vi "Launch Logger.vi"(8 "error in (no error)":errorcluster, 11 "Historian Module in":refnum<class "Historian Module.lvclass">) -> (0 "error out":errorcluster, 3 "Historian Module out":refnum<class "Historian Module.lvclass">)   [LabVIEW 2020, in "VolatusHistorian.lvlib" / "Historian Module.lvclass"]
uses:
  Historian Module.lvclass
  Historian Module.lvclass/Historian Module.ctl
  Volatus/Module/Module.lvclass
  Historian Logger/Historian Logger.lvclass
  C:/dev/lv20CE/relink/lv-volatus/Volatus/Module/Module.lvclass
  C:/dev/lv20CE/relink/lv-volatus/VolatusHistorian/Historian Module/Historian Module.lvclass
  VolatusConfig/Task/Task Config.lvclass
  C:/dev/lv20CE/relink/lv-volatus/VolatusConfig/VolatusConfigElement/VolatusConfigElement.lvclass
  C:/dev/lv20CE/relink/lv-volatus/VolatusConfig/Task/Task Config.lvclass
  C:/dev/lv20CE/relink/lv-volatus/VolatusHistorian/Historian Logger/Historian Logger.lvclass
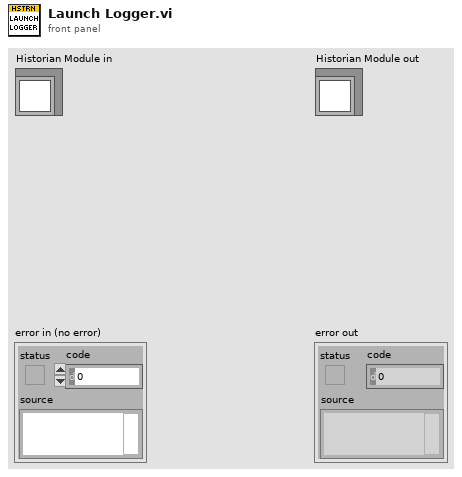
[diagram p1: front panel]
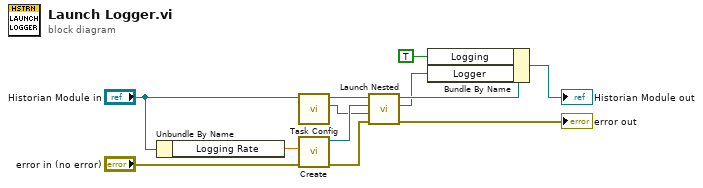
[diagram p0: block diagram]
diagram:
  n1 = Unbundle By Name("Historian Module in") -> ("Logging Rate"=w1:dbl)
  n2 = call "Task Config.vi"("Module in"="Historian Module in") -> ("Task Config"=w5:refnum<class "Task Config.lvclass">, "Module out"=w6:refnum<class "Historian Module.lvclass">)  [unwired: 8 in, 1 out]
  n3 = call "Create.vi"("error in (no error)"="error in (no error)", "Logging Rate"=w1) -> ("error out"=w7:errorcluster, "Historian Logger out"=w8:refnum<class "Historian Logger.lvclass">)  [unwired: 8 in]
  n4 = call "Launch Nested.vi"("error in (no error)"=w7, "Config Element"=w5, "Nested Module"=w8, "Parent in"=w6) -> ("error out"=→"error out":errorcluster, "MessageQ"=w9:refnum<class "MessageQ.lvclass">, "Parent out"=w11:refnum<class "Historian Module.lvclass">)  [unwired: 5 in]
  n5 = Bundle By Name(cluster=w11, "Logging"=TRUE ("Logger Used"), "Logger"=w9) -> (→"Historian Module out":refnum<class "Historian Module.lvclass">)
